vi "fake tool progress.vi"(8 "error in":errorcluster) -> (0 "error out":errorcluster, 2 "cancelled":bool, 3 "steps done":i32)   [LabVIEW 2020, in "MCP Server tests.lvlib"]
doc: "Test fixture tool: works through 10 steps of 200 ms. Before each step it calls Report Progress.vi with progress = step number, total 10 and message \"step n\", and stops as soon as cancelled? is TRUE. Afterwards it stores {\"steps\":n,\"cancelled\":..} in Progress Fixture Record.vi, n being the steps it finished. steps done and cancelled are its tool outputs."
uses:
  MCP Server tests.lvlib
  src/MCP Server/MCP Server.lvlib
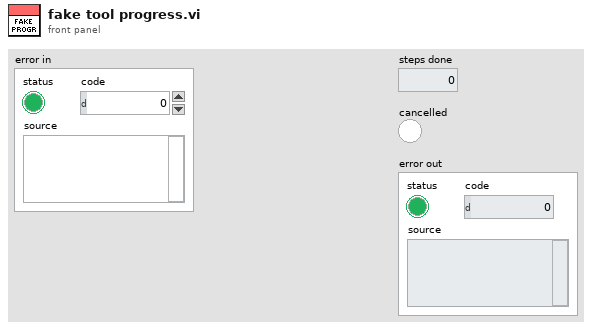
[diagram p1: front panel]
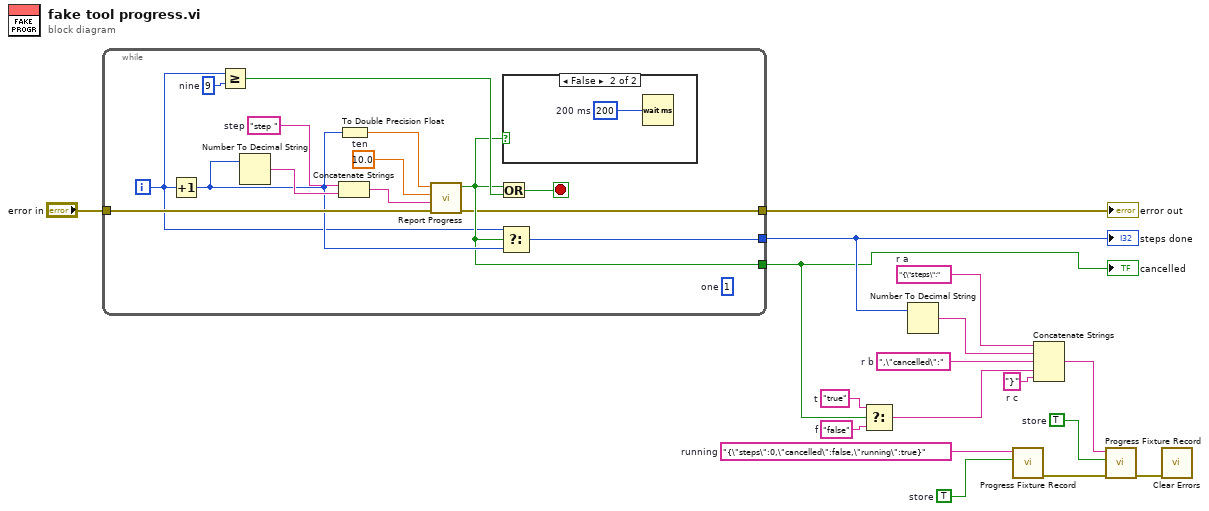
[diagram p0: block diagram]
diagram:
  w6 = TRUE  # store
  w8 = "}"  # r c
  w13 = "false"  # f
  w14 = "true"  # t
  w10 = ",\"cancelled\":"  # r b
  w12 = "{\"steps\":"  # r a
  w16 = TRUE  # store
  w17 = "{\"steps\":0,\"cancelled\":false,\"running\":true}"  # running
  n1 = while {
    tunnel: "error in" -> [w26]
    tunnel: [w21] -> w3
    tunnel: [w20] -> w2
    tunnel: [w19] -> w1
    i -> [w18]
    stop <- w22 stop-if-true
    w24 = 9  # nine
    w28 = 10.0  # ten
    w31 = "step "  # step
    (unwired) 1  # one
    n2 = Increment(x=w18) -> (x+1=w25:i32)
    n3 = Greater Or Equal?(x=w18, y=w24) -> (x >= y?=w23:bool)
    n4 = Number To Decimal String(number=w25) -> (decimal integer string=w30:string)  [unwired: 1 in]
    n5 = Concatenate Strings(w31, w30) -> (w27:string)
    n6 = To Double Precision Float(number=w25) -> (double precision float=w29:dbl)
    n7 = call "Report Progress.vi"("error in"=w26, "message"=w27, "total"=w28, "progress"=w29) -> ("error out"=w19:errorcluster, "cancelled?"=w20:bool)  [unwired: 6 in]
    n8 = Or(x=w20, y=w23) -> (x .or. y?=w22:bool)
    n9 = Select(t=w18, s=w20, f=w25) -> (s? t:f=w21:i32)
    n10 = case shown="False" w20 {
      frame True {
      }
      frame False {
        w32 = u32 200  # 200 ms
        n11 = Wait (ms)(milliseconds to wait=w32) -> ()  [unwired: 1 out]
      }
    }
  }
  "steps done" <- w3
  "cancelled" <- w2
  "error out" <- w1
  n12 = Select(t=w14, s=w2, f=w13) -> (s? t:f=w9:string)
  n13 = Number To Decimal String(number=w3) -> (decimal integer string=w11:string)  [unwired: 1 in]
  n14 = call "Progress Fixture Record.vi"("set?"=w16, "record in"=w17) -> ("error out"=w5:errorcluster)  [unwired: 8 in, 1 out]
  n15 = Concatenate Strings(w12, w11, w10, w9, w8) -> (w7:string)
  n16 = call "Progress Fixture Record.vi"("error in"=w5, "set?"=w6, "record in"=w7) -> ("error out"=w4:errorcluster)  [unwired: 7 in, 1 out]
  n17 = call <vilib>:"Clear Errors.vi"("error in (no error)"=w4) -> ()  [unwired: 5 in, 2 out]
